vi "RichToFlatauth_StartLoginRequest.vi"(5 "OutputClusterType":T1, 11 "InputCluster":T2) -> (3 "OutputCluster":T1)   [LabVIEW 2020, in "grpc-auth_client.lvlib"]
uses:
  grpc-auth_client.lvlib
  auth_StartLoginRequest.ctl
  auth_StartLoginRequest_Flat.ctl
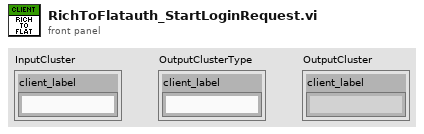
[diagram p1: front panel]
types:
  T1 = typedef "grpc-auth_client.lvlib/auth_StartLoginRequest_Flat.ctl" = cluster{"client_label":string}
  T2 = typedef "grpc-auth_client.lvlib/auth_StartLoginRequest.ctl" = cluster{"client_label":string}
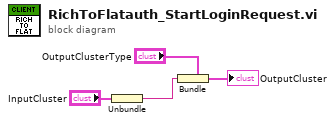
[diagram p0: block diagram]
diagram:
  n1 = Unbundle "Unbundle"("InputCluster") -> ("client_label"=w1:string)
  n2 = Bundle "Bundle"(cluster="OutputClusterType", "client_label"=w1) -> (→"OutputCluster":T1)
